vi "Open Library.vi"(6 "Library Path":path=path "", 8 "error in":errorcluster, 11 "Library Icon Data in":refnum<class "Library Icon Data.lvclass">) -> (0 "error out":errorcluster, 3 "Library Icon Data out":refnum<class "Library Icon Data.lvclass">)   [LabVIEW 2020, in "Library Icon Data.lvclass"]
doc: "Opens an Application reference and creates or opens the library at the given path."
uses:
  Library Icon Data.lvclass
  Library Icon Data.lvclass/Library Icon Data.ctl
  resource/plugins/lv_icon.lvlib
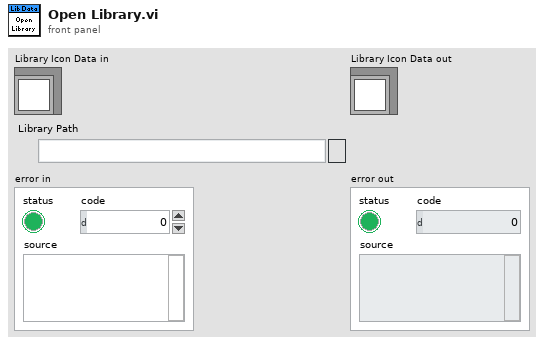
[diagram p1: front panel]
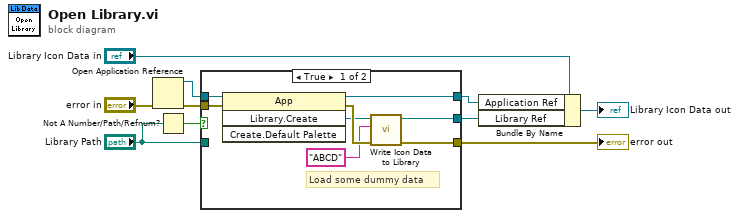
[diagram p0: block diagram]
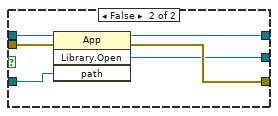
[diagram p2: hidden frame]
diagram:
  n1 = Open Application Reference(8:"error in") -> (0:w10:errorcluster, 3:w7:refnum<vi>)  [unwired: 3 in]
  n2 = Not A Number/Path/Refnum?(number/path/refnum="Library Path") -> (NaN/Path/Refnum?=w2:bool)
  n3 = case shown="True" w2 {
    tunnel: w10 -> [w18 w24]
    tunnel: [w16 w23] -> w8
    tunnel: w7 -> [w15 w22]
    tunnel: [w14 w21] -> w5
    tunnel: [w11 w20] -> w4
    tunnel: "Library Path" -> [_ w19]
    frame True {
      # "Load some dummy data"
      n4 = invoke class="App" method="Library.Create"(reference=w15, error in=w18) -> (reference out=w14:refnum<vi>, error out=w17:errorcluster, "Create Library"=w12:refnum<vi>)  [unwired: 2 in, 1 out]
      n5 = call "Write Icon Data to Library.vi"("error in"=w17, "Data"="ABCD", "Library Ref in"=w12) -> ("error out"=w16:errorcluster, "Library Ref out"=w11:refnum<vi>)  [unwired: 7 in]
    }
    frame False {
      n6 = invoke class="App" method="Library.Open"(reference=w22, error in=w24, "path"=w19) -> (reference out=w21:refnum<vi>, error out=w23:errorcluster, "Open Library"=w20:refnum<vi>)  [unwired: 1 in, 1 out]
    }
  }
  "error out" <- w8
  n7 = Bundle By Name(cluster="Library Icon Data in", "Application Ref"=w5, "Library Ref"=w4) -> (→"Library Icon Data out":refnum<class "Library Icon Data.lvclass">)
